vi "Connect.vi"(8 "error in (no error)":errorcluster, 10 "Connection":T1 {"Custom Data" format="%.0x"}, 11 "CIF_Iceoryx_BB":refnum<class "CIF_Iceoryx_BB.lvclass">) -> (0 "error out":errorcluster, 3 "CIF_Iceoryx_BB":refnum<class "CIF_Iceoryx_BB.lvclass">)   [LabVIEW 2021, in "CIF_Iceoryx_BB.lvclass"]
uses:
  CIF_Iceoryx_BB.lvclass
  ChannelCommon/typedef/New FIFO Instance Response.ctl
  D:/dev/Packages/CIF_Channels_Core/src/CIFChannels/CIFChannels.lvclass
  CIFChannels/CIFChannels.lvclass/CIFChannels.ctl
  CIF_Iceoryx_BB.lvclass/CIF_Iceoryx_BB.ctl
  ChannelCommon/typedef/Channel State.ctl
  <vilib>/CIF Foundation/CIF Iceoryx/typedef/Topic Full Names.ctl
  CIF_Iceoryx_Chan/Typedef/Iceoryx Channel Error.ctl
  Accessors/Write Reader Reference.vi
  CIFChannels/Accessors/Read Name.vi
  CIFChannels/Accessors/Read Direction.vi
  CIFChannels/Accessors/Read Pattern.vi
  CIF_Iceoryx_Chan/SubVIs/Iceoryx Channel Errors Core.vi
  ChannelCommon/ChannelCommon.lvlib
  CIFChannels/CIFChannels.lvclass
  <vilib>/CIF Foundation/CIF Iceoryx/Iceoryx.lvlib
  CIF_Iceoryx_Chan/CIF_Iceoryx_Chn.lvclass
  Iceorxy Utilities/Iceoryx Channel Utilities.lvlib
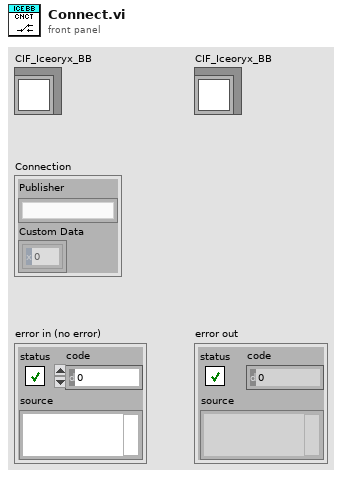
[diagram p1: front panel]
types:
  T1 = typedef "ChannelCommon.lvlib/New FIFO Instance Response.ctl" = cluster{"Publisher":string, "Custom Data":u8[]}
  T2 = typedef "ChannelCommon.lvlib/Channel State.ctl" = enum8{"Creating", "Disconnected", "Connecting", "Connected", "Destroyed"}
  T3 = typedef "Iceoryx.lvlib/Topic Full Names.ctl" = cluster{"BlackBoard":string, "Topic":string, "Type Override":string}
  T4 = typedef "CIF_Iceoryx_Chn.lvclass/Iceoryx Channel Error.ctl" = enum16{"Type Mismatch", "Name Mismatch", "Override Required"}
  T5 = typedef "ChannelCommon.lvlib/Direction.ctl" = enum8{"Publisher", "Subscriber"}
  T6 = typedef "ChannelCommon.lvlib/Channel Pattern.ctl" = enum8{"Unknown", "Tag", "FIFO", "MultiFIFO", "BackpressureFIFO"}
  T7 = typedef "Iceoryx.lvlib/BB Reader Refnum.ctl" = cluster{"refnum":u64, "BB Reader":enum8{"bb_reader"}}
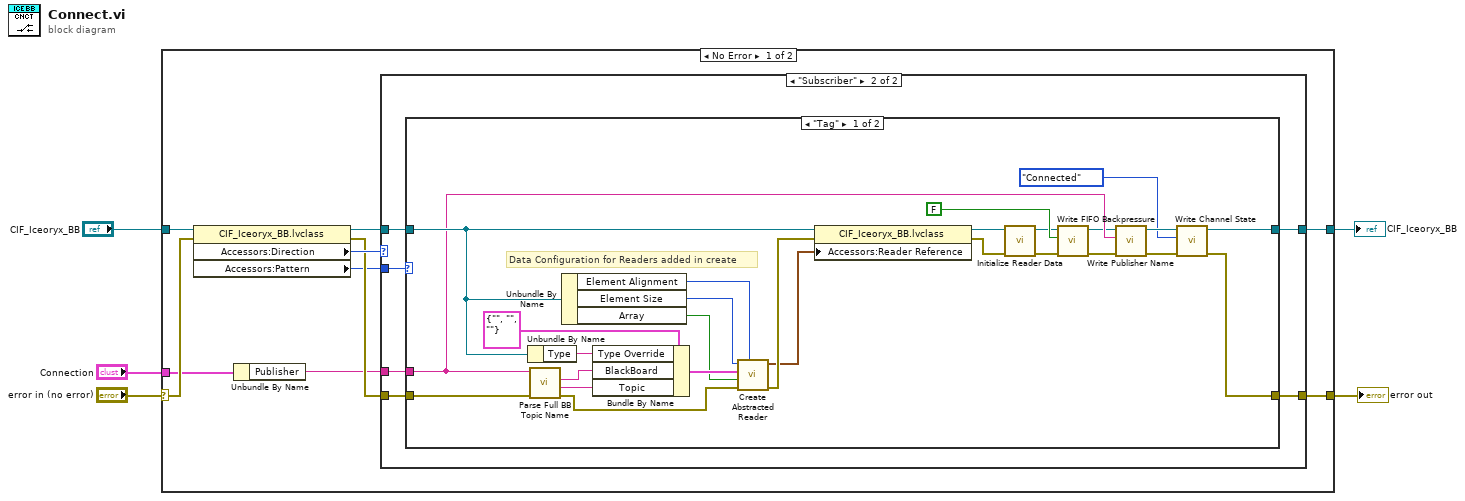
[diagram p0: block diagram]
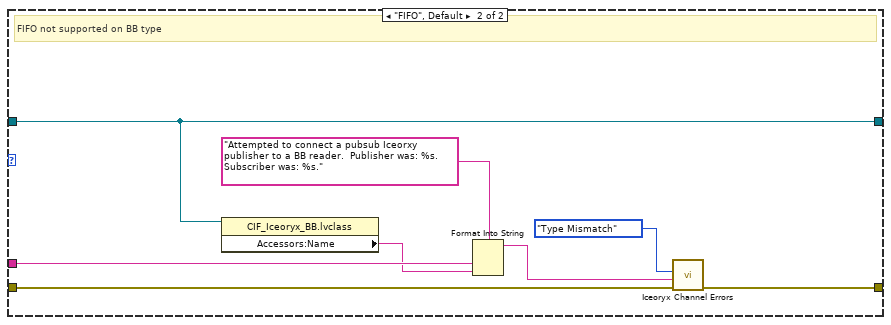
[diagram p3: hidden frame]
diagram:
  n1 = case shown="No Error" "error in (no error)" {
    selector: "error in (no error)" -> [w15 w59]
    tunnel: [w10 w59] -> w4
    tunnel: [w12 w58] -> w1
    tunnel: "CIF_Iceoryx_BB" -> [w6 w58]
    tunnel: "Connection" -> [w9 _]
    frame No Error {
      n2 = property class="CIF_Iceoryx_BB.lvclass"(reference=w6, error in=w15) -> (reference out=w14:refnum<class "CIF_Iceoryx_BB.lvclass">, error out=w11:errorcluster, "Accessors:Direction"=w13:T5, "Accessors:Pattern"=w7:T6)
      n3 = Unbundle By Name(w9) -> ("Publisher"=w8:string)
      n4 = case shown="\"Subscriber\"" w13 {
        tunnel: w14 -> [w17 w21]
        tunnel: [w17 w20] -> w12
        tunnel: w11 -> [w16 w23]
        tunnel: w8 -> [_ w22]
        tunnel: [w16 w19] -> w10
        tunnel: w7 -> [_ w18]
        frame "Publisher" {
          # "No connection step needed for publishers"
        }
        frame "Subscriber" {
          n5 = case shown="\"Tag\"" w18 {
            tunnel: w23 -> [w37 w56]
            tunnel: w22 -> [w39 w54]
            tunnel: w21 -> [w42 w52]
            tunnel: [w32 w52] -> w20
            tunnel: [w31 w55] -> w19
            frame "Tag" {
              # "Data Configuration for Readers added in create"
              n6 = Unbundle By Name(w42) -> ("Type"=w47:string)
              n7 = call "Parse Full BB Topic Name.vi"("error in"=w37, "Full BB Topic Name"=w39) -> ("error out"=w36:errorcluster, "Topic"=w38:string, "Blackboard name"=w35:string)  [unwired: 6 in, 1 out]
              n8 = Unbundle By Name(w42) -> ("Element Alignment"=w45:u32, "Element Size"=w44:u32, "Array"=w43:bool)
              n9 = Bundle By Name(cluster=T3 {"BlackBoard"="", "Topic"="", "Type Override"=""} ("Topic Name"), "Type Override"=w47, "BlackBoard"=w35, "Topic"=w38) -> (w46:T3)
              n10 = call <vilib>:"Create Abstracted Reader.vi"("Element Alignment"=w45, "error in (no error)"=w36, "Array"=w43, "Topic Name"=w46, "Element Size"=w44) -> ("error out"=w41:errorcluster, "Reader Reference"=w34:T7)  [unwired: 5 in]
              n11 = property class="CIF_Iceoryx_BB.lvclass"(reference=w42, error in=w41, "Accessors:Reader Reference"=w34) -> (reference out=w33:refnum<class "CIF_Iceoryx_BB.lvclass">, error out=w40:errorcluster)
              n12 = call-dynamic "Initialize Reader Data.vi"("error in (no error)"=w40, "CIF_Iceoryx_BB in"=w33) -> ("error out"=w29:errorcluster, "CIF_Iceoryx_BB out"=w30:refnum<class "CIF_Iceoryx_BB.lvclass">)  [unwired: 8 in]
              n13 = call "Write FIFO Backpressure.vi"("error in (no error)"=w29, "Backpressure"=FALSE, "CIFChannels in"=w30) -> ("error out"=w27:errorcluster, "CIFChannels out"=w28:refnum<class "CIF_Iceoryx_BB.lvclass">)  [unwired: 7 in]
              n14 = call "Write Publisher Name.vi"("error in (no error)"=w27, "Publisher Name"=w39, "CIFChannels in"=w28) -> ("error out"=w25:errorcluster, "CIFChannels out"=w26:refnum<class "CIF_Iceoryx_BB.lvclass">)  [unwired: 7 in]
              n15 = call "Write Channel State.vi"("error in (no error)"=w25, "Channel State"=Channel_State."Connected", "CIFChannels in"=w26) -> ("error out"=w31:errorcluster, "CIFChannels out"=w32:refnum<class "CIF_Iceoryx_BB.lvclass">)  [unwired: 7 in]
            }
            frame "FIFO", Default {
              # "FIFO not supported on BB type"
              n16 = property class="CIF_Iceoryx_BB.lvclass"(reference=w52) -> ("Accessors:Name"=w50:string)  [unwired: 1 in, 2 out]
              n17 = Format Into String(format string="Attempted to connect a pubsub Iceorxy publisher to a BB reader.  Publisher was: %s. Subscriber was: %s." ("String to Append"), w54, w50) -> (resulting string=w53:string)  [unwired: 2 in, 1 out]
              n18 = call "Iceoryx Channel Errors.vi"("error in (no error)"=w56, "String to Append"=w53, "Error"=Iceoryx_Channel_Error."Type Mismatch") -> ("error out"=w55:errorcluster)  [unwired: 8 in]
            }
          }
        }
      }
    }
    frame Error {
    }
  }
  "error out" <- w4
  "CIF_Iceoryx_BB" <- w1
